vi "RFH-test-excel_converter.vi"() -> ()   [LabVIEW 2020]
doc: "Test panel, run by hand: converts an R140 Excel file with RFH-convert-r140 and plots the result. The user picks the file and the destination folder."
uses:
  RFH-Reflection_File_Handler.lvlib
panel:
  out "Frequency 2":dbl[](array[numeric])
  out "Frequency":dbl[][](graph)
  out "Frequency":dbl[](array[numeric])
  out "Imag":T1(graph)
  out "Real":T2(graph)
  in  "Destination Folder":path
  in  "file path":path
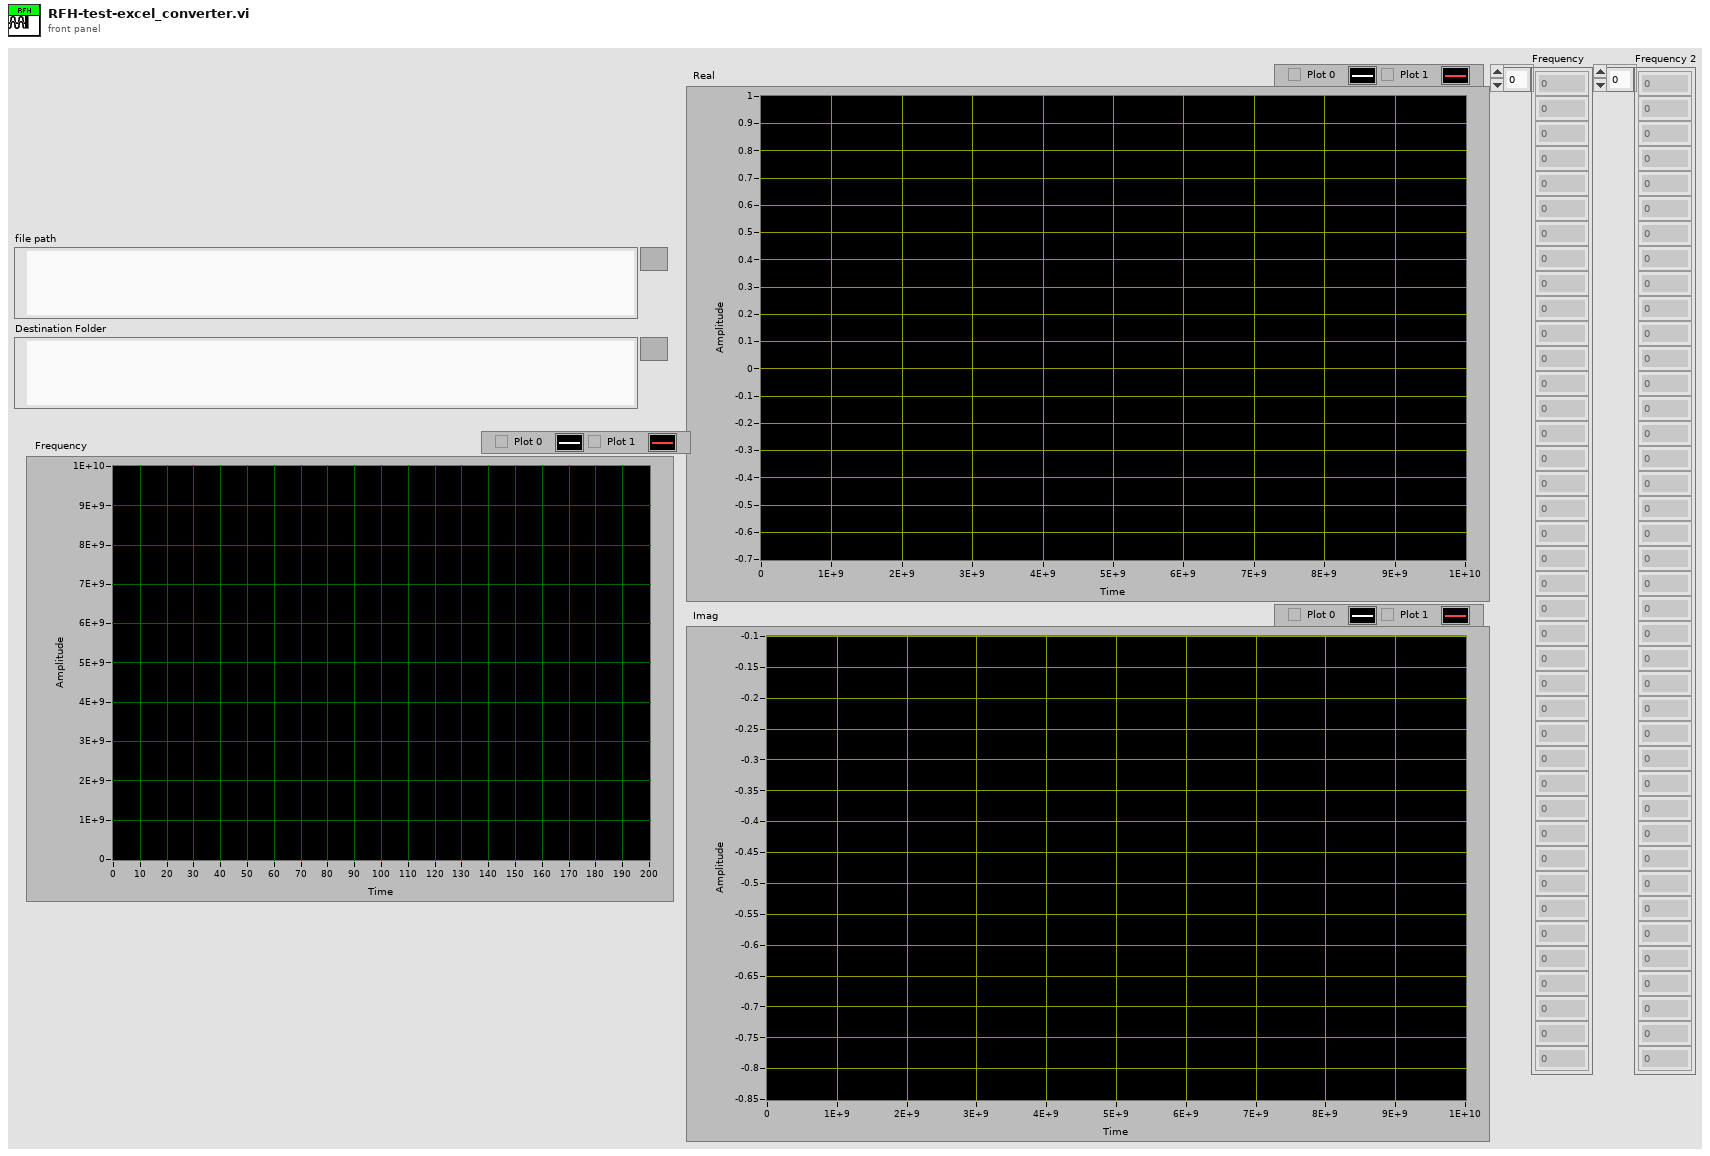
[diagram p1: front panel]
types:
  T1 = cluster{"Frequency":dbl[], "Reflection''":dbl[]}[]
  T2 = cluster{"Frequency":dbl[], "Reflection'":dbl[]}[]
  T3 = typedef "RFH-Reflection_File_Handler.lvlib/RFH-common_data_format.ctl" = cluster{"Frequency":dbl[], "Reflection'":dbl[], "Reflection''":dbl[], "Permativity'":dbl[], "Permativity''":dbl[], "Conductivity":dbl[], "Loss Tangent":dbl[], "Resistance":dbl[], "Reactance":dbl[]}
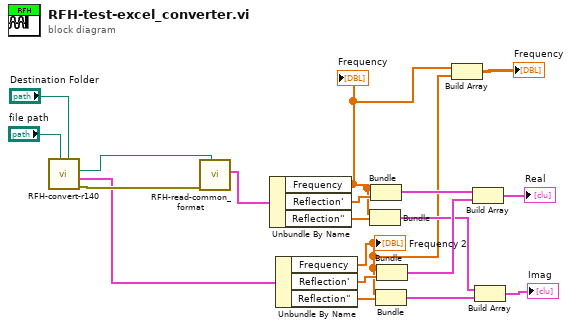
[diagram p0: block diagram]
diagram:
  n1 = call "RFH-convert-r140.vi"("Destination Folder"="Destination Folder", "file path"="file path") -> ("error out"=w18:errorcluster, "Data"=w15:T3, "converted file path"=w19:path)  [unwired: 7 in]
  n2 = call "RFH-read-common_format.vi"("file path (dialog if empty)"=w19, "error in"=w18) -> ("Common Format"=w10:T3)  [unwired: 8 in, 1 out]
  n3 = Unbundle By Name(w10) -> ("Frequency"=w2:dbl[], "Reflection'"=w11:dbl[], "Reflection''"=w12:dbl[])
  "Frequency" <- w2
  n4 = Unbundle By Name(w15) -> ("Frequency"=w3:dbl[], "Reflection'"=w14:dbl[], "Reflection''"=w13:dbl[])
  "Frequency 2" <- w3
  n5 = Bundle("Frequency"=w2, "Reflection''"=w12) -> (w6:cluster{"Frequency":dbl[], "Reflection''":dbl[]})  [unwired: 1 in]
  n6 = Bundle("Frequency"=w2, "Reflection'"=w11) -> (w9:cluster{"Frequency":dbl[], "Reflection'":dbl[]})  [unwired: 1 in]
  n7 = Bundle("Frequency"=w3, "Reflection''"=w13) -> (w7:cluster{"Frequency":dbl[], "Reflection''":dbl[]})  [unwired: 1 in]
  n8 = Bundle("Frequency"=w3, "Reflection'"=w14) -> (w8:cluster{"Frequency":dbl[], "Reflection'":dbl[]})  [unwired: 1 in]
  n9 = Build Array(w2, w3) -> (→"Frequency":dbl[][])
  n10 = Build Array(w9, w8) -> (→"Real":T2)
  n11 = Build Array(w6, w7) -> (→"Imag":T1)
